vi "Init.vi"(8 "Error In":errorcluster caption="错误输入", 10 "Time and Data In":T1, 11 "Sample Settings In":T2={"设备信息"={"初始索引子集"=[], "模拟信号采集通道"="Dev1", "数字-供电"="", "数字-光控"="", "光控设备"="", "光电设备分离？"=FALSE, "光谱保存路径"=path "", "环数"=0}, "测量控制"={"测头拿起"=FALSE, "起始保存"=FALSE, "测头供电"=TRUE, "测头出光"=TRUE}, "测量"={"每波长测量次数"=5, "波长"=[0, 0, 0, 0, 0, 0], "起始周期"=1, "起始测量周期"=0}, "等待"={"等待时间(s)"=0.0, "等待方式"=FALSE, "每x周期/点等待"=8, "等待时"=enum."无电无光"}, "校准"={"暗电流校准值初值"=[], "温度校准值"=[0.0, 0.0, 0.0, 0.0, 0.0, 0.0, 0.00013, 0.00013, 0.00013, 0.00013, 0.00013, 0.00013], "校准模式"=enum."逐周期"}, "图表相关"={"文件-时间"=""}, "CSM"={"CSM Name"=""}}) -> (0 "Error Out":errorcluster caption="错误输出", 2 "Time and Data Out":T1, 3 "Sample Settings Out":T2={"设备信息"={"初始索引子集"=[], "模拟信号采集通道"="Dev1", "数字-供电"="", "数字-光控"="", "光控设备"="", "光电设备分离？"=FALSE, "光谱保存路径"=path "", "环数"=0}, "测量控制"={"测头拿起"=FALSE, "起始保存"=FALSE, "测头供电"=TRUE, "测头出光"=TRUE}, "测量"={"每波长测量次数"=5, "波长"=[0, 0, 0, 0, 0, 0], "起始周期"=1, "起始测量周期"=0}, "等待"={"等待时间(s)"=0.0, "等待方式"=FALSE, "每x周期/点等待"=8, "等待时"=enum."无电无光"}, "校准"={"暗电流校准值初值"=[], "温度校准值"=[0.0, 0.0, 0.0, 0.0, 0.0, 0.0, 0.00013, 0.00013, 0.00013, 0.00013, 0.00013, 0.00013], "校准模式"=enum."逐周期"}, "图表相关"={"文件-时间"=""}, "CSM"={"CSM Name"=""}})   [LabVIEW 2026, in "UI-无创.lvlib" / "Acquisition.lvlib"]
uses:
  Acquisition.lvlib
  Supports/Sample Settings.ctl
  Supports/Time and Data_OP.ctl
  <vilib>/DAQmx/create/channels.llb/DAQmx Create Channel (DO-Digital Output).vi
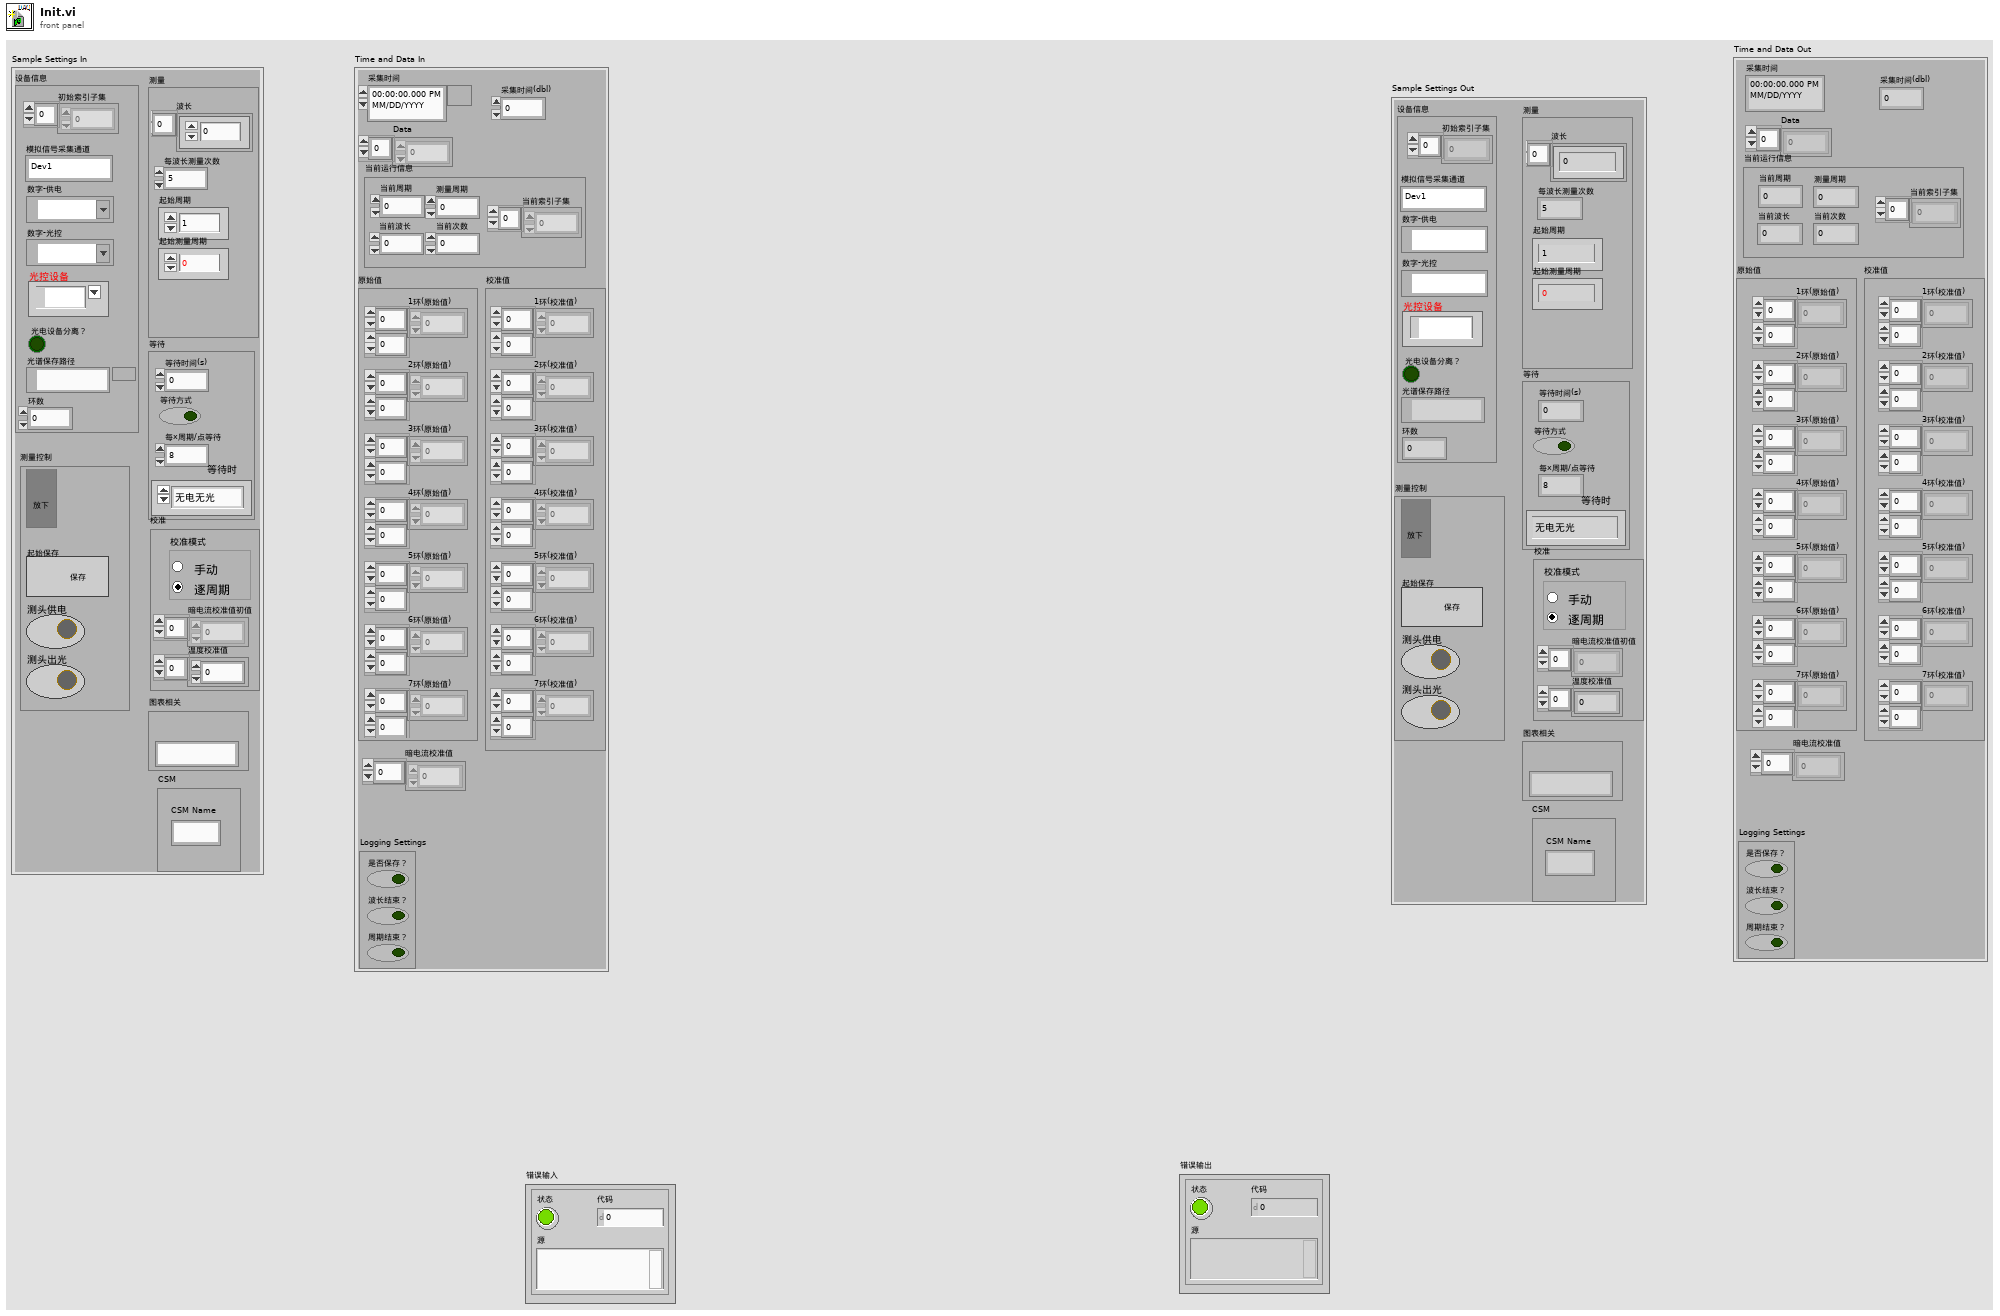
[diagram p1: front panel]
types:
  T1 = typedef "UI-无创.lvlib/Time and Data_OP.ctl" = cluster{"采集时间":timestamp, "采集时间(dbl)":dbl, "Data":dbl[], "当前运行信息":cluster{"当前周期":i32, "当前次数":i32, "测量周期":i32, "当前索引子集":i8[], "当前波长":i32}, "暗电流校准值":dbl[], "Logging Settings":cluster{"是否保存？":bool, "波长结束？":bool, "周期结束？":bool}, "原始值":cluster{"1环(原始值)":dbl[][], "2环(原始值)":dbl[][], "3环(原始值)":dbl[][], "4环(原始值)":dbl[][], "5环(原始值)":dbl[][], "6环(原始值)":dbl[][], "7环(原始值)":dbl[][]}, "校准值":cluster{"1环(校准值)":dbl[][], "2环(校准值)":dbl[][], "3环(校准值)":dbl[][], "4环(校准值)":dbl[][], "5环(校准值)":dbl[][], "6环(校准值)":dbl[][], "7环(校准值)":dbl[][]}}
  T2 = typedef "UI-无创.lvlib/Sample Settings.ctl" = cluster{"设备信息":cluster{"初始索引子集":i8[], "模拟信号采集通道":string, "数字-供电":refnum<k21>, "数字-光控":refnum<k21>, "光控设备":tag, "光电设备分离？":bool, "光谱保存路径":path, "环数":u8}, "测量控制":cluster{"测头拿起":bool, "起始保存":bool, "测头供电":bool, "测头出光":bool}, "测量":cluster{"每波长测量次数":i32, "波长":i32[], "起始周期":i32, "起始测量周期":i32}, "等待":cluster{"等待时间(s)":dbl, "等待方式":bool, "每x周期/点等待":i32, "等待时":enum16{"无电无光", "有电无光", "无电有光", "有电有光"}}, "校准":cluster{"暗电流校准值初值":dbl[], "温度校准值":dbl[], "校准模式":T3}, "图表相关":cluster{"文件-时间":string}, "CSM":cluster{"CSM Name":string}}
  T3 = typedef "UI-无创.lvlib/暗电流校准模式.ctl" = enum32{"手动", "逐周期"}
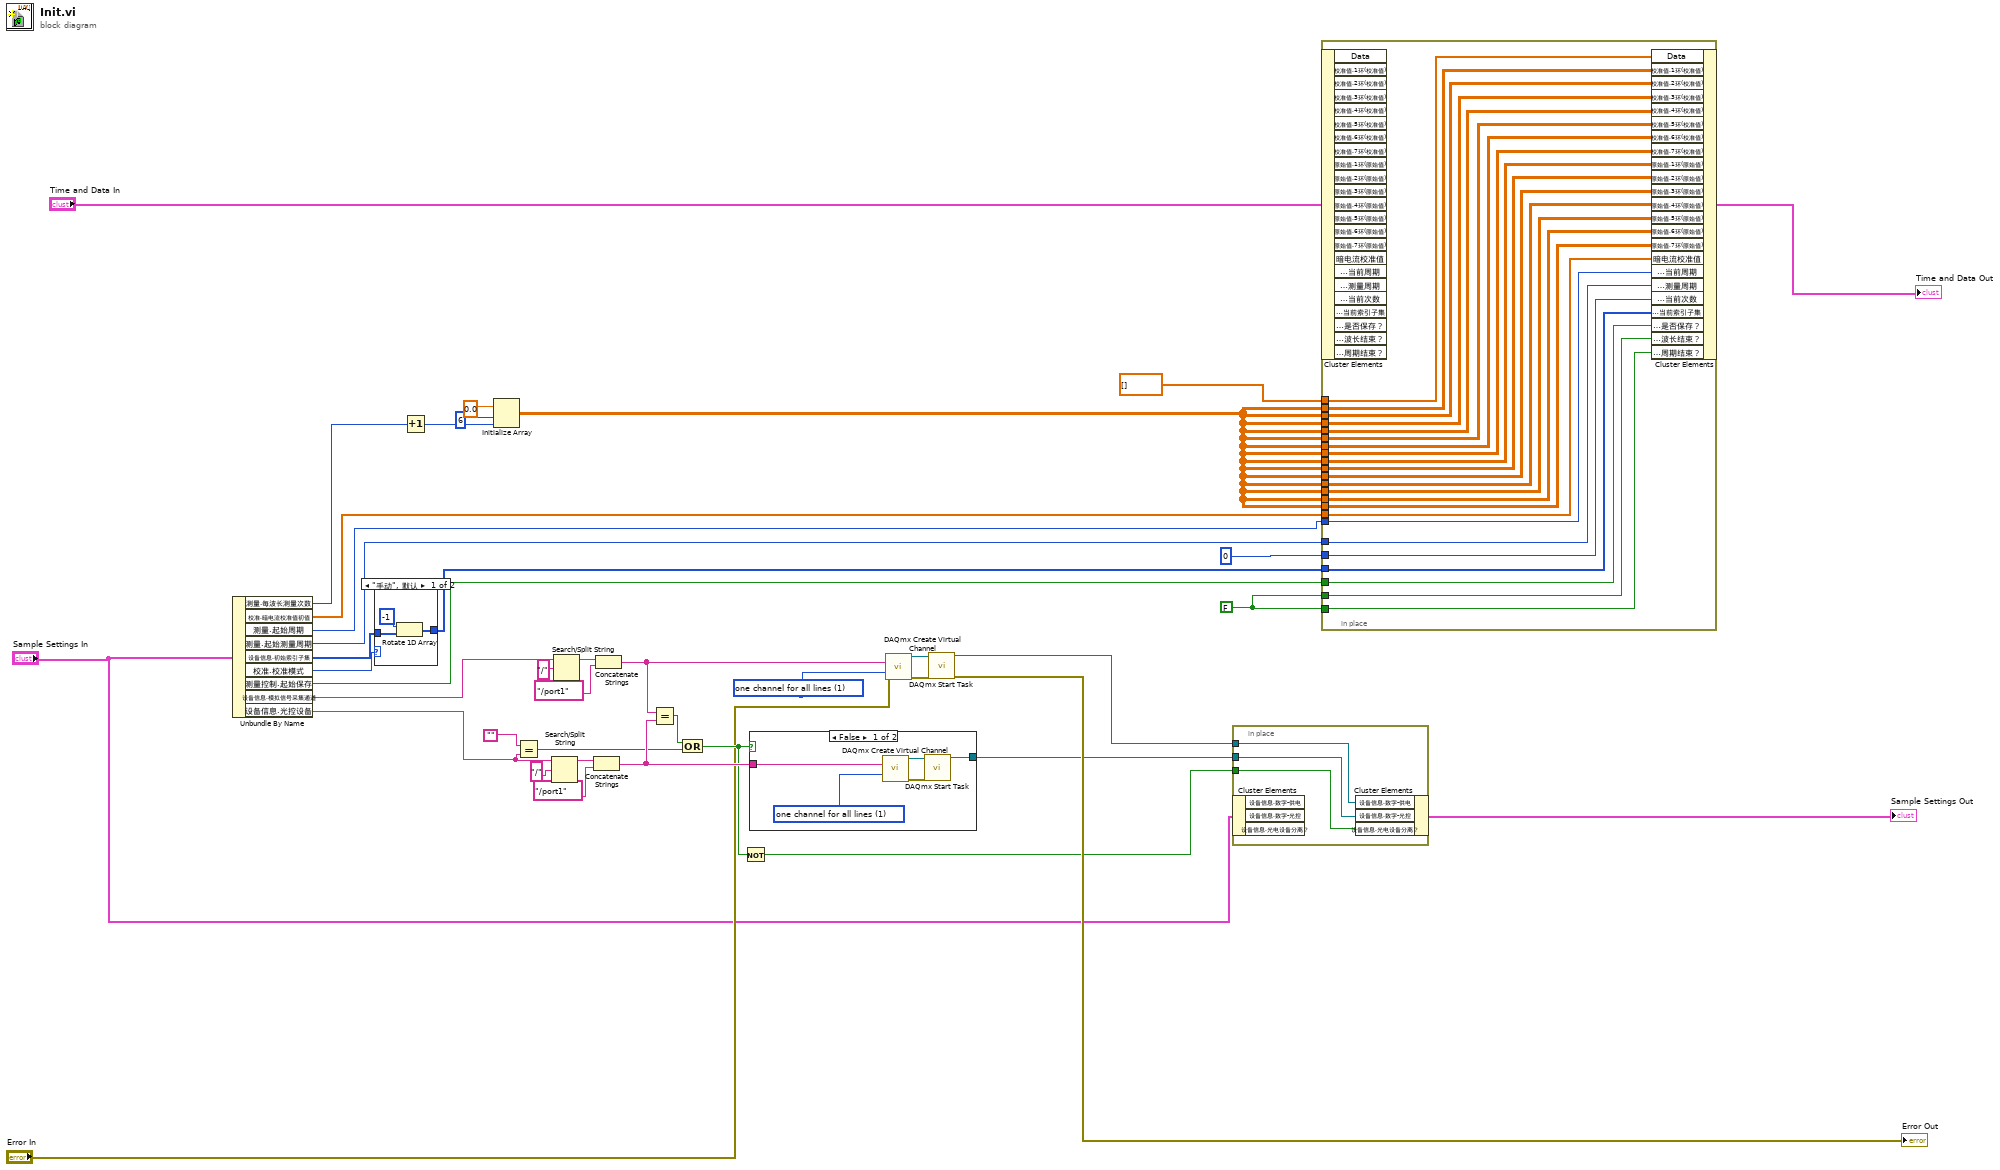
[diagram p0: block diagram]
diagram:
  w10 = FALSE
  w39 = 1 items=["one channel for each line", "one channel for all lines"] ("line grouping")
  n1 = Unbundle By Name("Sample Settings In") -> ("测量.每波长测量次数"=w22:i32, "校准.暗电流校准值初值"=w15:dbl[], "测量.起始周期"=w14:i32, "测量.起始测量周期"=w13:i32, "设备信息.初始索引子集"=w3:i8[], "校准.校准模式"=w2:T3, "测量控制.起始保存"=w11:bool, "设备信息.模拟信号采集通道"=w21:string, "设备信息.光控设备"=w26:tag)
  n2 = case shown="\"手动\", 默认" w2 {
    tunnel: w3 -> [w43 w45]
    tunnel: [w42 w45] -> w1
    frame "手动", Default {
      n3 = Rotate 1D Array(1:w43, 2:-1 ("n")) -> (0:w42:i8[])
    }
    frame "逐周期" {
    }
  }
  n4 = Increment(x=w22) -> (x+1=w24:i32)
  n5 = Initialize Array(0.0, 6 ("维数大小"), w24) -> (w16:dbl[][])
  n6 = Equal?(x="", y=w26) -> (x = y?=w27:bool)
  n7 = Search/Split String(string=w26, search string/char (-)="/" ("搜索字符串/字符(-)")) -> (substring before match=w34:string)  [unwired: 1 in, 2 out]
  n8 = Search/Split String(string=w21, search string/char (-)="/" ("搜索字符串/字符(-)")) -> (substring before match=w37:string)  [unwired: 1 in, 2 out]
  n9 = Concatenate Strings(w34, "/port1" ("字符串")) -> (w31:string)
  n10 = Concatenate Strings(w37, "/port1" ("字符串")) -> (w32:string)
  n11 = Equal?(x=w32, y=w31) -> (x = y?=w28:bool)
  n12 = Compound Arithmetic op=OR(w28, w27) -> (w29:bool)
  n13 = Not(x=w29) -> (.not. x?=w4:bool)
  n14 = case shown="False" w29 {
    tunnel: w31 -> [w47 w51]
    tunnel: [w46 w51] -> w5
    frame False {
      w50 = 1 items=["one channel for each line", "one channel for all lines"] ("line grouping")
      n15 = call-poly <vilib>:"DAQmx Create Virtual Channel.vi"("lines"=w47, "line grouping"=w50) -> ("task out"=w49:refnum<k21>, "error out"=w48:errorcluster)  [unwired: 12 in]
      n16 = call <vilib>:"DAQmx Start Task.vi"("task/channels in"=w49, "error in"=w48) -> ("task out"=w46:refnum<k21>)  [unwired: 12 in, 1 out]
    }
    frame True {
    }
  }
  n17 = call-poly <vilib>:"DAQmx Create Virtual Channel.vi"("lines"=w32, "line grouping"=w39, "error in"="Error In") -> ("task out"=w40:refnum<k21>, "error out"=w41:errorcluster)  [unwired: 11 in]
  n18 = call <vilib>:"DAQmx Start Task.vi"("task/channels in"=w40, "error in"=w41) -> ("task out"=w6:refnum<k21>, "error out"=→"Error Out":errorcluster)  [unwired: 12 in]
  n19 = in-place {
    in-place-border: w6 -> [w54]
    in-place-border: w5 -> [w53]
    in-place-border: w4 -> [w52]
    n20 = in-place-cluster #1("Sample Settings In") -> ()  [unwired: 3 out]
    n21 = in-place-cluster #1("设备信息.数字-供电"=w54, "设备信息.数字-光控"=w53, "设备信息.光电设备分离？"=w52) -> (→"Sample Settings Out":T2)
  }
  n22 = in-place {
    in-place-border: dbl[] [] ("Data") -> [w77]
    in-place-border: w16 -> [w76]
    in-place-border: w16 -> [w75]
    in-place-border: w16 -> [w74]
    in-place-border: w16 -> [w73]
    in-place-border: w16 -> [w72]
    in-place-border: w16 -> [w71]
    in-place-border: w16 -> [w70]
    in-place-border: w16 -> [w69]
    in-place-border: w16 -> [w68]
    in-place-border: w16 -> [w67]
    in-place-border: w16 -> [w66]
    in-place-border: w16 -> [w65]
    in-place-border: w16 -> [w64]
    in-place-border: w16 -> [w63]
    in-place-border: w15 -> [w62]
    in-place-border: w14 -> [w61]
    in-place-border: w13 -> [w60]
    in-place-border: 0 ("当前运行信息.当前次数") -> [w59]
    in-place-border: w1 -> [w58]
    in-place-border: w11 -> [w57]
    in-place-border: w10 -> [w56]
    in-place-border: w10 -> [w55]
    n23 = in-place-cluster #2("Time and Data In") -> ()  [unwired: 23 out]
    n24 = in-place-cluster #2("Data"=w77, "校准值.1环(校准值)"=w76, "校准值.2环(校准值)"=w75, "校准值.3环(校准值)"=w74, "校准值.4环(校准值)"=w73, "校准值.5环(校准值)"=w72, "校准值.6环(校准值)"=w71, "校准值.7环(校准值)"=w70, "原始值.1环(原始值)"=w69, "原始值.2环(原始值)"=w68, "原始值.3环(原始值)"=w67, "原始值.4环(原始值)"=w66, "原始值.5环(原始值)"=w65, "原始值.6环(原始值)"=w64, "原始值.7环(原始值)"=w63, "暗电流校准值"=w62, "当前运行信息.当前周期"=w61, "当前运行信息.测量周期"=w60, "当前运行信息.当前次数"=w59, "当前运行信息.当前索引子集"=w58, "Logging Settings.是否保存？"=w57, "Logging Settings.波长结束？"=w56, "Logging Settings.周期结束？"=w55) -> (→"Time and Data Out":T1)
  }
